vi "Main.vi"() -> ()   [LabVIEW 2019]
doc: "The myRIO Project template acquires acceleration data from the onboard accelerometer and displays the changes of acceleration values in a waveform chart."
uses:
  <vilib>/myRIO/Common/Instrument Driver Framework/myRIO v1.0/Encoder/typedefs/Encoder Count Direction Enum.ctl
  <vilib>/myRIO/Common/Instrument Driver Framework/myRIO v1.0/Encoder/typedefs/Encoder Signal Mode.ctl
  <vilib>/myRIO/Common/Instrument Driver Framework/myRIO v1.0/Encoder/typedefs/Encoder Channels Enum.ctl
  <vilib>/myRIO/Common/Instrument Driver Framework/Utilities/typedefs/Generic FPGA Reference.ctl
  <vilib>/myRIO/Common/Instrument Driver Framework/Utilities/typedefs/myRIO v1.0 Reference.ctl
  <vilib>/myRIO/Common/Instrument Driver Framework/Utilities/typedefs/Hardware Version Enum.ctl
  <vilib>/myRIO/Common/Instrument Driver Framework/Utilities/typedefs/myRIO Generic Hardware Reference.ctl
  <vilib>/myRIO/Instrument Drivers/Onboard IO/Encoder/typedefs/Encoder Reference.ctl
  <vilib>/myRIO/Instrument Drivers/Onboard IO/Encoder/Encoder.lvlib
  <vilib>/myRIO/Instrument Drivers/Onboard IO/Encoder/vis/Read.vi
  <vilib>/myRIO/Common/Instrument Driver Framework/myRIO v1.0/Encoder/typedefs/Encoder Configuration v1.0.ctl
  <vilib>/userDefined/High Color/nirio_resource_hc.ctl
  <vilib>/myRIO/Common/Instrument Driver Framework/myRIO v1.0/Encoder/vis/myRIO v1.1 Open Encoder.vi
  <vilib>/myRIO/Common/Instrument Driver Framework/myRIO v1.0/Encoder/vis/myRIO v1.0 Configure Encoder.vi
  <vilib>/myRIO/Instrument Drivers/Onboard IO/Encoder/vis/myRIO Encoder Open.xnode
  <vilib>/myRIO/Common/Instrument Driver Framework/Utilities/vis/Is FPGA Ref Available.vi
  <vilib>/myRIO/Express VI/Onboard IO/Encoder/Encoder Express VI.xnode
  <vilib>/ptbypt/NI_PtbyPt.lvlib
  <vilib>/myRIO/Instrument Drivers/Onboard IO/PWM/typedefs/PWM Configuration.ctl
  <vilib>/myRIO/Instrument Drivers/Onboard IO/PWM/PWM.lvlib
  <vilib>/myRIO/Common/Instrument Driver Framework/myRIO v1.0/PWM/typedefs/PWM Channels Enum.ctl
  <vilib>/myRIO/Instrument Drivers/Onboard IO/PWM/typedefs/PWM Reference.ctl
  <vilib>/myRIO/Instrument Drivers/Onboard IO/PWM/vis/Set Duty Cycle and Frequency.vi
  <vilib>/myRIO/Common/Instrument Driver Framework/myRIO v1.0/PWM/vis/myRIO v1.1 Open PWM.vi
  <vilib>/myRIO/Instrument Drivers/Onboard IO/PWM/vis/myRIO PWM Open.xnode
  <vilib>/myRIO/Express VI/Onboard IO/PWM/PWM Express VI.xnode
  <vilib>/myRIO/Common/Instrument Driver Framework/myRIO v1.0/DIO/typedefs/DIO Channels Enum.ctl
  <vilib>/myRIO/Common/Instrument Driver Framework/myRIO v1.0/DIO/typedefs/DIO Channels List.ctl
  <vilib>/myRIO/Instrument Drivers/Onboard IO/DIO/typedefs/DIO Reference.ctl
  <vilib>/myRIO/Instrument Drivers/Onboard IO/DIO/DIO.lvlib
  <vilib>/myRIO/Instrument Drivers/Onboard IO/DIO/vis/Write.vi
  <vilib>/myRIO/Common/Instrument Driver Framework/myRIO v1.0/DIO/vis/myRIO v1.1 Open DIO.vi
  <vilib>/myRIO/Instrument Drivers/Onboard IO/DIO/vis/myRIO DIO Open.xnode
  <vilib>/myRIO/Express VI/Onboard IO/DO/DO Express VI.xnode
  <vilib>/addons/control/pid/NI_PID_pid.lvlib
  <vilib>/addons/control/pid/pid.llb/PID (DBL).vi
  <vilib>/myRIO/Common/Instrument Driver Framework/myRIO v1.0/Accelerometer/typedefs/Accelerometer Channels Enum.ctl
  <vilib>/myRIO/Common/Instrument Driver Framework/myRIO v1.0/Accelerometer/typedefs/Accelerometer Channels List.ctl
  <vilib>/myRIO/Instrument Drivers/Onboard Devices/Accelerometer/typedefs/Accelerometer Reference.ctl
  <vilib>/myRIO/Instrument Drivers/Onboard Devices/Accelerometer/Accelerometer.lvlib
  <vilib>/myRIO/Instrument Drivers/Onboard Devices/Accelerometer/vis/Read.vi
  <vilib>/myRIO/Instrument Drivers/Onboard Devices/Accelerometer/vis/myRIO Accelerometer Open.xnode
  <vilib>/myRIO/Express VI/Onboard Devices/Accelerometer/Accelerometer Express VI.xnode
  <vilib>/myRIO/Instrument Drivers/Utilities/Utilities.lvlib
  <vilib>/Utility/file.llb/Write Delimited Spreadsheet (DBL).vi
  <vilib>/myRIO/Common/Instrument Driver Framework/myRIO v1.0/Accelerometer/vis/myRIO v1.1 Open Accelerometer.vi
panel:
  out "Velocidad M2":dbl
  out "Velocidad  M1":dbl
  out "Aporte de FF-M1":dbl
  out "Aporte de FF-M2":dbl
  out "Distancia M2":dbl
  out "Distancia  M1":dbl
  in  "T pasa-bajos":dbl=0.1
  in  "zona_muerta (°)":dbl=2.5
  out "aX_grav":dbl
  in  "KgR_sub":dbl=0.18 format="%#_13g"
  in  "KgR_baj":dbl=0.11 format="%#_13g"
  in  "KgL_baj":dbl=0.12 format="%#_13g"
  in  "KgL_sub":dbl=0.19 format="%#_13g"
  in  "Offset acel_X":dbl=-0.114
  in  "ang_rampa":dbl=10.0
  out "Inclinación X":dbl
  in  "Offset_acel_Y":dbl
  out "Inclinación Y":dbl
  out "Duty Cycle calculado":dbl
  out "Duty Cycle enviado":dbl
  out "roll_n":dbl
  out "pitch_n":dbl
  out "Verifica si se guardo csv":errorcluster
  out "Verifica si se guardo csv 2":errorcluster
  out "error out 2":errorcluster
  out "RPM M1":dbl
  out "RPM GAUGE M1":dbl(knob) scale=0.0..100.0
  out "Dirección de Giro M1":enum16{"Counting Up", "Counting Down"}(ring)
  out "Cuentas M1 (Der)":dbl
  out "Posición angular M1":dbl(knob) scale=-360.0..360.0
  out "Posición M1":dbl
  out "Frecuencia (rev/s)":dbl
  out "Vueltas Dadas M1":dbl
  out "Posición angular M2":dbl(knob) scale=-360.0..360.0
  out "Dirección de Giro M2":enum16{"Counting Up", "Counting Down"}(ring)
  out "Posición M2":dbl
  out "RPM GAUGE M2":dbl(knob) scale=0.0..100.0
  out "Vueltas Dadas M2":dbl
  out "RPM M2":dbl
  out "Cuentas M2 (Izq)":dbl
  in  "Referencia M1 y M2":dbl
  in  "Velocidad":dbl
  in  "v(cm/s)":dbl
  in  "w (rad/s)":dbl
  in  "PWM Manual":dbl
  out "a_encoder":dbl
  out "a_enc_f":dbl
  out "aX_f":dbl
  out "aY_f":dbl
  out "aZ_f":dbl
  out "phi":dbl
  out "phi_deg":dbl
  out "periodo real (seg)":dbl
  in  "Ref Platfform Movement":dbl
  in  "ROBOT MÓVIL CON PLATAFORMA DE BALANCEO - GRUPO 2":T1(tab)
  in  "?":bool
  in  "Tipo de referencia":enum16{"Sinusoidal", "Constante"}(ring)
  out "Coordenada xy vs t":cluster{dbl, dbl, "Referencia":dbl}(graph)
  out "Angulos de servos":cluster{dbl, dbl}(graph)
  out "Recepción del UART":string
  in  "PID EJE Y":T2={"proportional gain (Kc)"=0.14897, "integral time (Ti, min)"=0.03, "derivative time (Td, min)"=0.004327} {"derivative time (Td, min)" format="%.6f"; "integral time (Ti, min)" format="%.6f"; "proportional gain (Kc)" format="%.6f"}
  in  "PID EJE X":T2={"proportional gain (Kc)"=0.1164, "integral time (Ti, min)"=0.03, "derivative time (Td, min)"=0.005282} {"derivative time (Td, min)" format="%.6f"; "integral time (Ti, min)" format="%.6f"; "proportional gain (Kc)" format="%.6f"}
  in  "Frecuencia (Hz)":dbl=50.0
  in  "Modo de operación":enum16{"Platform movement", "Ball Control"}(ring)=enum."Ball Control"
  in  "dt (s)":dbl=0.0167 format="%.4f"
  in  "Tipo de control":enum16{"SMC", "LQR", "PID"}(ring)=enum."PID"
  in  "Eje":enum16{"xy", "y", "x", "Home"}(ring)
  in  "Referencia Control":dbl
  in  "Rango Salida Y":cluster{"output high":dbl, "output low":dbl}={"output high"=25.0, "output low"=-25.0} {"output low" format="%.2f"; "output high" format="%.2f"}
  in  "Rango Salida X":cluster{"output high":dbl, "output low":dbl}={"output high"=25.0, "output low"=-25.0} {"output low" format="%.2f"; "output high" format="%.2f"}
  out "Saturación (inclinación de plataforma)":cluster{dbl, dbl}(graph)
  in  "Longitud de brazo [mm]":dbl=35.0
  in  "R (L/2) [mm]":dbl=59.0
  out "Roll -  Eje X":dbl
  out "Pitch - Eje Y":dbl
  out "Error Ángulo (°)":dbl
  out "Error Distancia (cm)":dbl
  out "LLEGÓ":bool
  out "Avanzando":bool
  out "Girando":bool
  in  "Tolerancia (cm)":dbl=0.3
  out "Recorrido Eje X (cm)":dbl
  out "SIGUE Vel M2":bool
  out "SIGUE Vel M1":bool
  out "Comportamiento de ángulos (°)":cluster{"phi_lim":dbl, "roll_lim":dbl}(graph)
  out "Control Lazo Interno":cluster{"f":dbl, dbl, "f":dbl, dbl}(graph)
  in  "Movimiento":T3(ring)=enum."Recta"
  in  "INICIAR MOTORES":bool
  in  "STOP ALL":bool
  in  "Referencia":dbl=220.0
  in  "REINICIAR":bool caption="Reiniciar cuentas"
  in  "PI - M1":T2={"proportional gain (Kc)"=0.014853, "integral time (Ti, min)"=0.000665, "derivative time (Td, min)"=0.0} {"derivative time (Td, min)" format="%.6f"; "integral time (Ti, min)" format="%.6f"; "proportional gain (Kc)" format="%.6f"}
  in  "PI - M2":T2={"proportional gain (Kc)"=0.01026, "integral time (Ti, min)"=0.000604, "derivative time (Td, min)"=0.0} {"derivative time (Td, min)" format="%.6f"; "integral time (Ti, min)" format="%.6f"; "proportional gain (Kc)" format="%.6f"}
  out "Señal de control de Velocidades":cluster{"output":dbl, "output":dbl}(graph)
  out "Lazo externo - Posición":cluster{"x":dbl, "y":dbl}(graph)={"x"=50.0, "y"=49.66663306165075}
  out "Lazo externo - Rumbo":cluster{"x":dbl, "y":dbl}(graph)
  in  "MODO CONTROL":T4(ring)=enum."Trayectoria"
  out "Móvil dt":dbl=0.01
  out "X (cm)":dbl
  out "Y (cm)":dbl
  out "theta (deg)":dbl
  in  "Kd":dbl=1.38 format="%#_13g"
  in  "Ky":dbl=0.048 format="%#_13g"
  in  "Kth":dbl=1.38 format="%#_13g"
  in  "Tol cm/s":dbl=1.5
  out "Falla M2":bool
  out "Falla M1":bool
  in  "Rango Salida PWM":cluster{"output high":dbl, "output low":dbl}={"output high"=1.0, "output low"=-1.0} {"output low" format="%.2f"; "output high" format="%.2f"}
  out "Desvio en Y (cm)":cluster{"y":dbl}(graph)
  out "Giro Realizado (°)":dbl
  # "Filtro Pasa - Bajo"
  # "Lectura - Lazo Interno"
  # "Lectura - Lazo Externo"
  # "Feed-Forward"
  # "CONTROL PID DE CADA EJE -  PLATAFORMA DE BALANCEO"
  # "Reinicio"
  # "CONTROL DE TRAYECTORIA EN CASCADA - BASE MÓVIL"
  # "Operación y Seguridad"
  # "Modo de Control - Lazo Interno"
  # "Modo de Control - Lazo Externo"
  # "ODOMETRÍA"
  # "GANANCIAS - LAZO EXTERNO"
  # "ERROR Y LLEGADA"
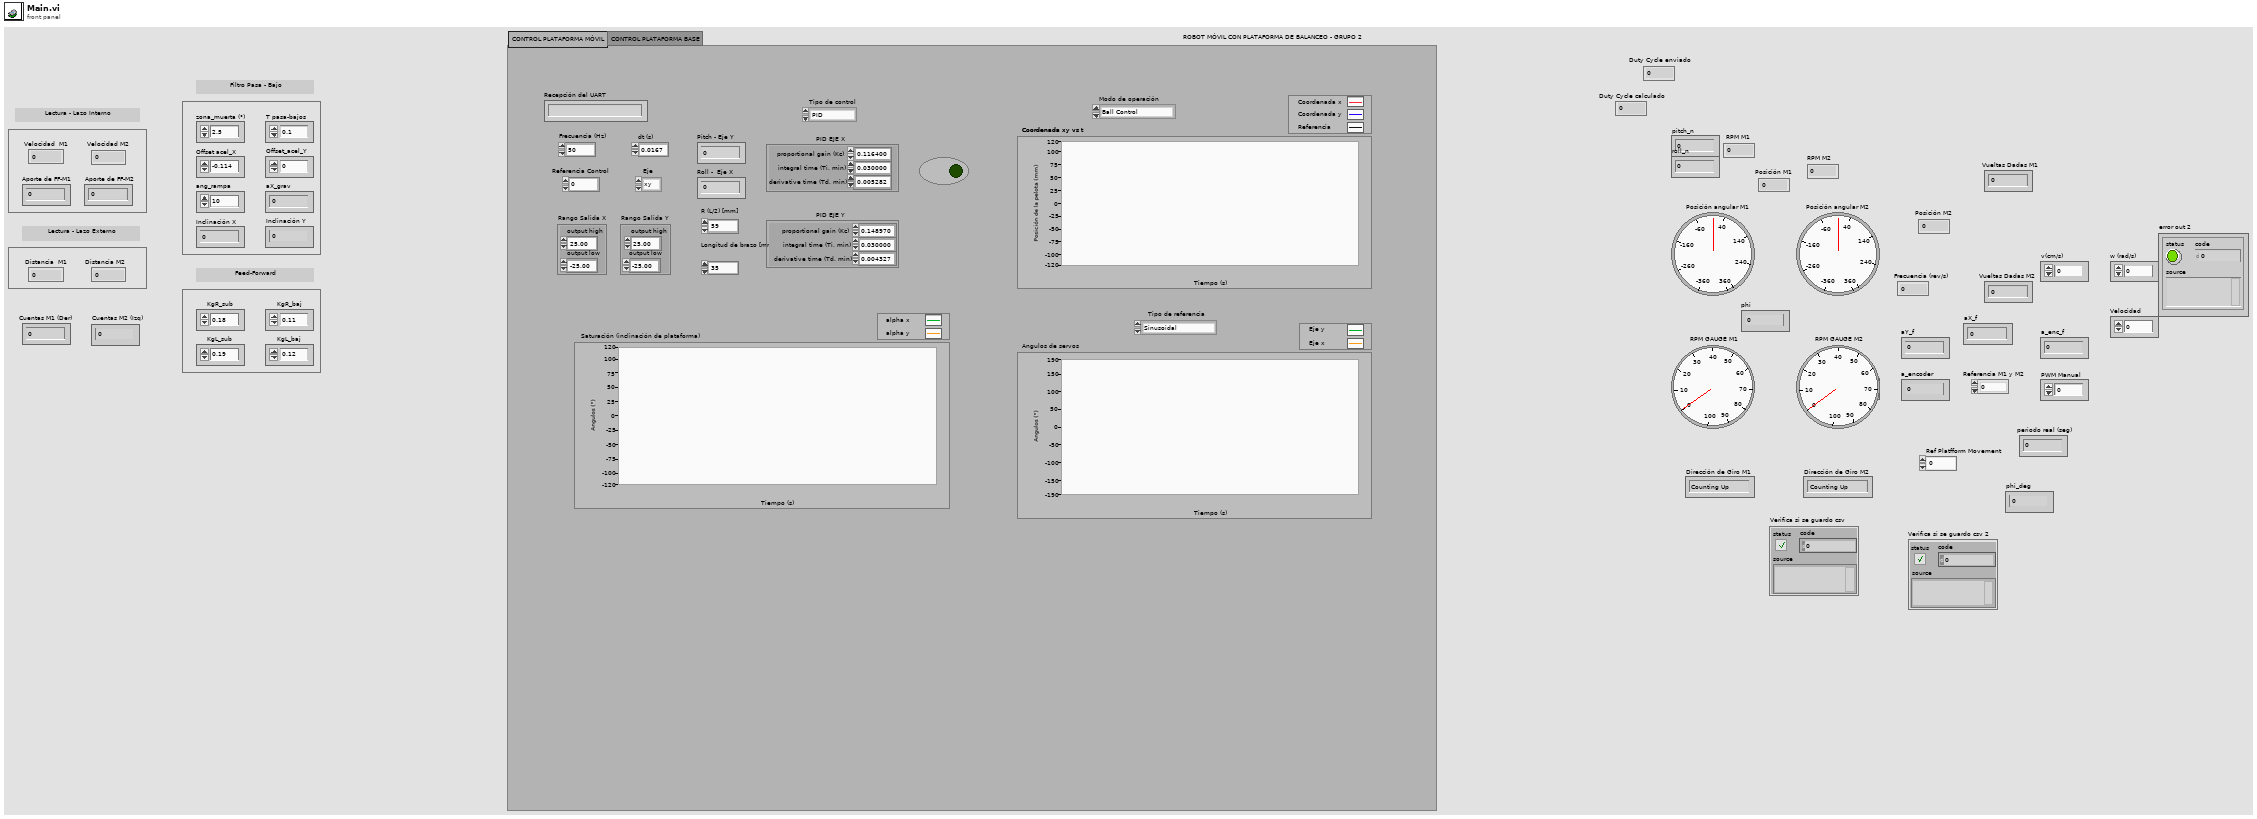
[diagram p1: front panel]
types:
  T1 = enum32{"CONTROL PLATAFORMA MÓVIL", "CONTROL PLATAFORMA BASE"}
  T2 = cluster{"proportional gain (Kc)":dbl, "integral time (Ti, min)":dbl, "derivative time (Td, min)":dbl}
  T3 = enum16{"Manual", "Recta", "Giro centro", "Giro rueda fija", "Rutina Piso", "Ida y Vuelta", "Rutina Rampa", ""}
  T4 = enum16{"Identificación", "Lazo Interno", "Trayectoria"}
  T5 = typedef "PWM.lvlib/PWM Reference.ctl" = cluster{"myRIO Reference":T6, "PWM Channels Enum":T10, "PWM Configuration":T11}
  T6 = typedef "myRIO Generic Hardware Reference.ctl" = cluster{"myRIO Model":T7, "myRIO Hardware Reference":T8}
  T7 = typedef "Hardware Version Enum.ctl" = enum16{"Unknown", "myRIO-1900", "myRIO-1950", "roboRIO", "NI ELVIS RIO CM", "ELVIS III"}
  T8 = typedef "myRIO v1.0 Reference.ctl" = cluster{"Generic FPGA Reference":T9, "Allow multiple opens":bool}
  T9 = typedef "Generic FPGA Reference.ctl" = refnum<k20>
  T10 = typedef "PWM Channels Enum.ctl" = enum16{"Not Connected", "C/PWM0", "C/PWM1", "A/PWM0", "A/PWM1", "A/PWM2", "A/PWM3", "A/PWM4", "A/PWM5", "A/PWM6", "A/PWM7", "A/PWM8", "A/PWM9", "A/PWM10", "A/PWM11", "A/PWM12", "A/PWM13", "A/PWM14", "A/PWM15", "A/PWM16", "A/PWM17", "A/PWM18", "A/PWM19", "B/PWM0", "B/PWM1", "B/PWM2", "B/PWM3", "B/PWM4", "B/PWM5", "B/PWM6", "B/PWM7", "B/PWM8", "B/PWM9", "B/PWM10", "B/PWM11", "B/PWM12", "B/PWM13", "B/PWM14", "B/PWM15", "B/PWM16", "B/PWM17", "B/PWM18", "B/PWM19", "PWM/PWM0", "PWM/PWM1", "PWM/PWM2", "PWM/PWM3", "PWM/PWM4", "PWM/PWM5", "PWM/PWM6", "PWM/PWM7", "PWM/PWM8", "PWM/PWM9"}
  T11 = typedef "PWM.lvlib/PWM Configuration.ctl" = cluster{"Frequency":dbl, "Duty Cycle":dbl}
  T12 = typedef "nirio_resource_hc.ctl" = tag
  T13 = enum16{"Identificación", "Lazo Interno", "Trayectoria", ""}
  T14 = typedef "Accelerometer.lvlib/Accelerometer Reference.ctl" = cluster{"myRIO Reference":T6, "Accelerometer Channels List":T15, "LSB Weight":dbl}
  T15 = typedef "Accelerometer Channels List.ctl" = T16[]
  T16 = typedef "Accelerometer Channels Enum.ctl" = enum16{"Not Connected", "X-Axis", "Y-Axis", "Z-Axis"}
  T17 = typedef "DIO.lvlib/DIO Reference.ctl" = cluster{"myRIO Reference":T6, "DIO Channels List":T18}
  T18 = typedef "DIO Channels List.ctl" = T19[]
  T19 = typedef "DIO Channels Enum.ctl" = enum16{"Not Connected", "C/DIO0", "C/DIO1", "C/DIO2", "C/DIO3", "C/DIO4", "C/DIO5", "C/DIO6", "C/DIO7", "A/DIO0", "A/DIO1", "A/DIO2", "A/DIO3", "A/DIO4", "A/DIO5", "A/DIO6", "A/DIO7", "A/DIO8", "A/DIO9", "A/DIO10", "A/DIO11", "A/DIO12", "A/DIO13", "A/DIO14", "A/DIO15", "A/DIO16", "A/DIO17", "A/DIO18", "A/DIO19", "B/DIO0", "B/DIO1", "B/DIO2", "B/DIO3", "B/DIO4", "B/DIO5", "B/DIO6", "B/DIO7", "B/DIO8", "B/DIO9", "B/DIO10", "B/DIO11", "B/DIO12", "B/DIO13", "B/DIO14", "B/DIO15", "B/DIO16", "B/DIO17", "B/DIO18", "B/DIO19", "LED0", "LED1", "LED2", "LED3", "Button0", "DIO/DIO0", "DIO/DIO1", "DIO/DIO2", "DIO/DIO3", "DIO/DIO4", "DIO/DIO5", "DIO/DIO6", "DIO/DIO7", "DIO/DIO8", "DIO/DIO9", "SPI/CS0", "SPI/CS1", "SPI/CS2", "SPI/CS3", "LED RADIO (Green)", "LED RADIO (Red)", "LED COMM (Green)", "LED COMM (Red)", "LED MODE (Green)", "LED MODE (Red)"}
  T20 = typedef "Encoder.lvlib/Encoder Reference.ctl" = cluster{"myRIO Reference":T6, "Encoder Channels Enum":T21}
  T21 = typedef "Encoder Channels Enum.ctl" = enum16{"Not Connected", "C/ENC0", "C/ENC1", "A/ENC", "A/ENC0", "A/ENC1", "A/ENC2", "A/ENC3", "A/ENC4", "A/ENC5", "A/ENC6", "A/ENC7", "A/ENC8", "A/ENC9", "B/ENC", "B/ENC0", "B/ENC1", "B/ENC2", "B/ENC3", "B/ENC4", "B/ENC5", "B/ENC6", "B/ENC7", "B/ENC8", "B/ENC9", "DIO/ENC0", "DIO/ENC1", "DIO/ENC2", "DIO/ENC3", "DIO/ENC4"}
  T22 = typedef "Encoder Signal Mode.ctl" = enum16{"Quadrature phase signal", "Step and direction signal"}
  T23 = enum16{"open", "replace", "create", "open or create", "replace or create", "replace or create with confirmation"}
  T24 = typedef "Encoder Count Direction Enum.ctl" = enum16{"Counting Up", "Counting Down"}
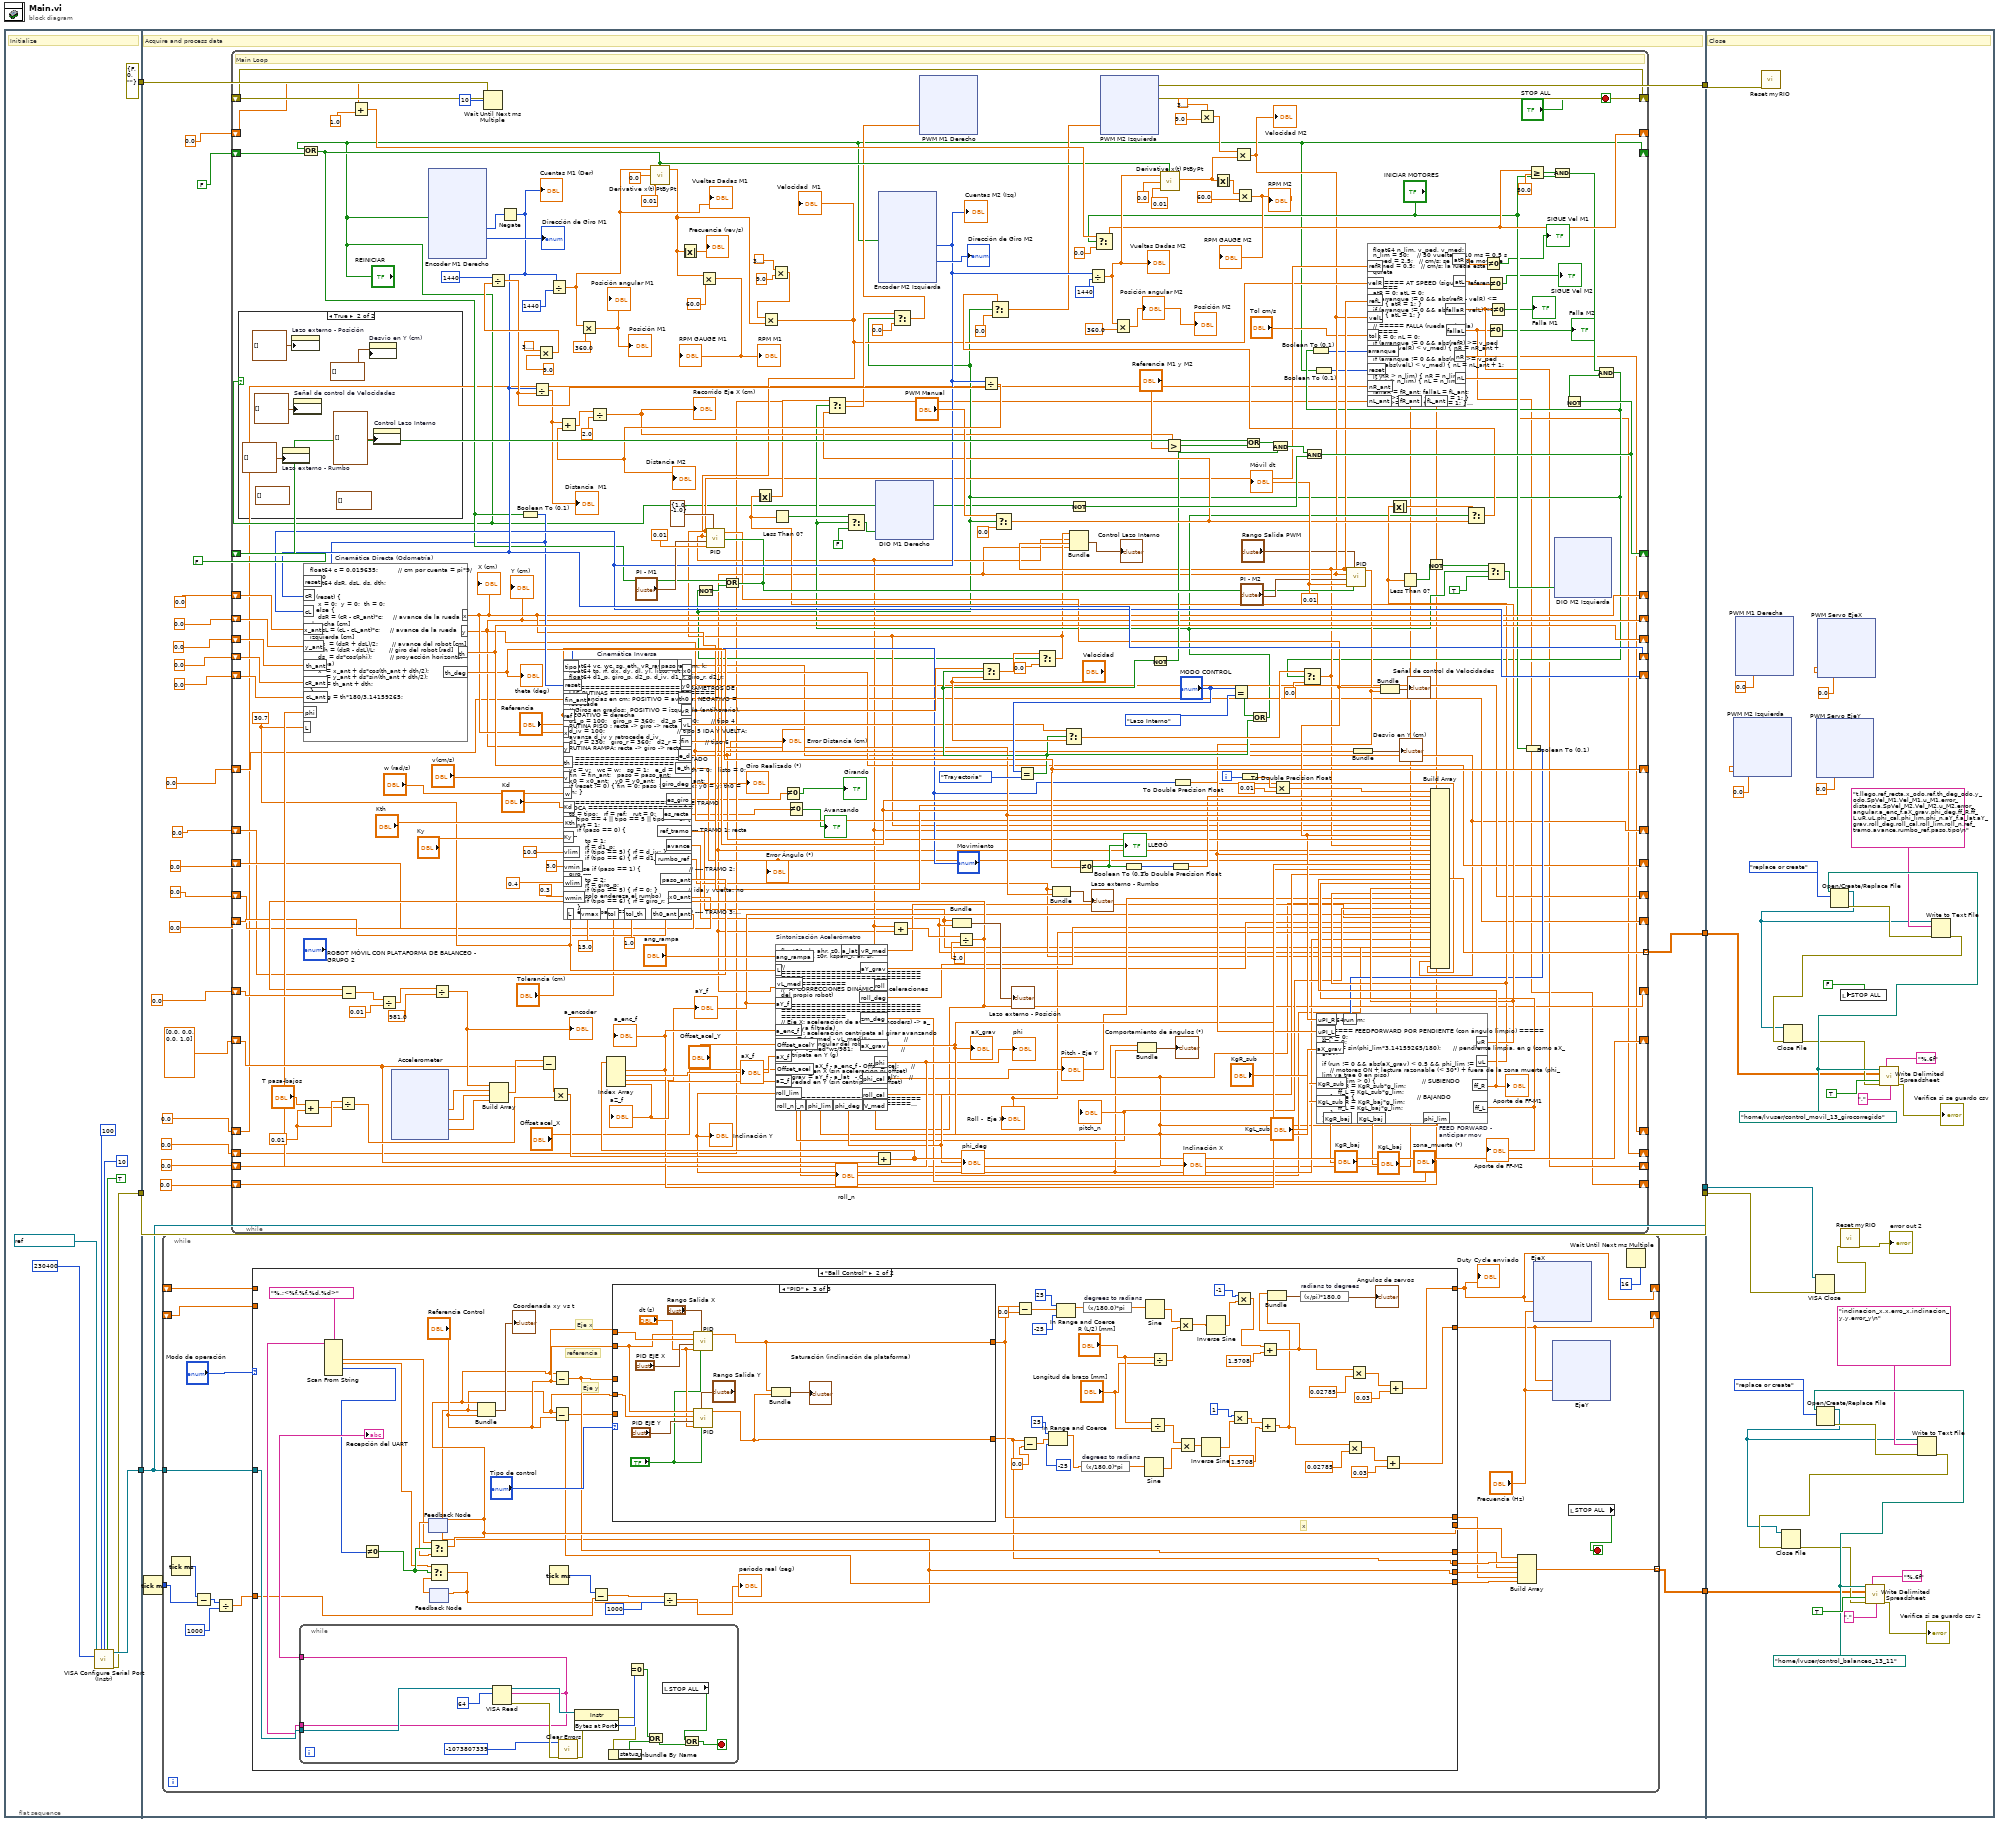
[diagram p0: block diagram]
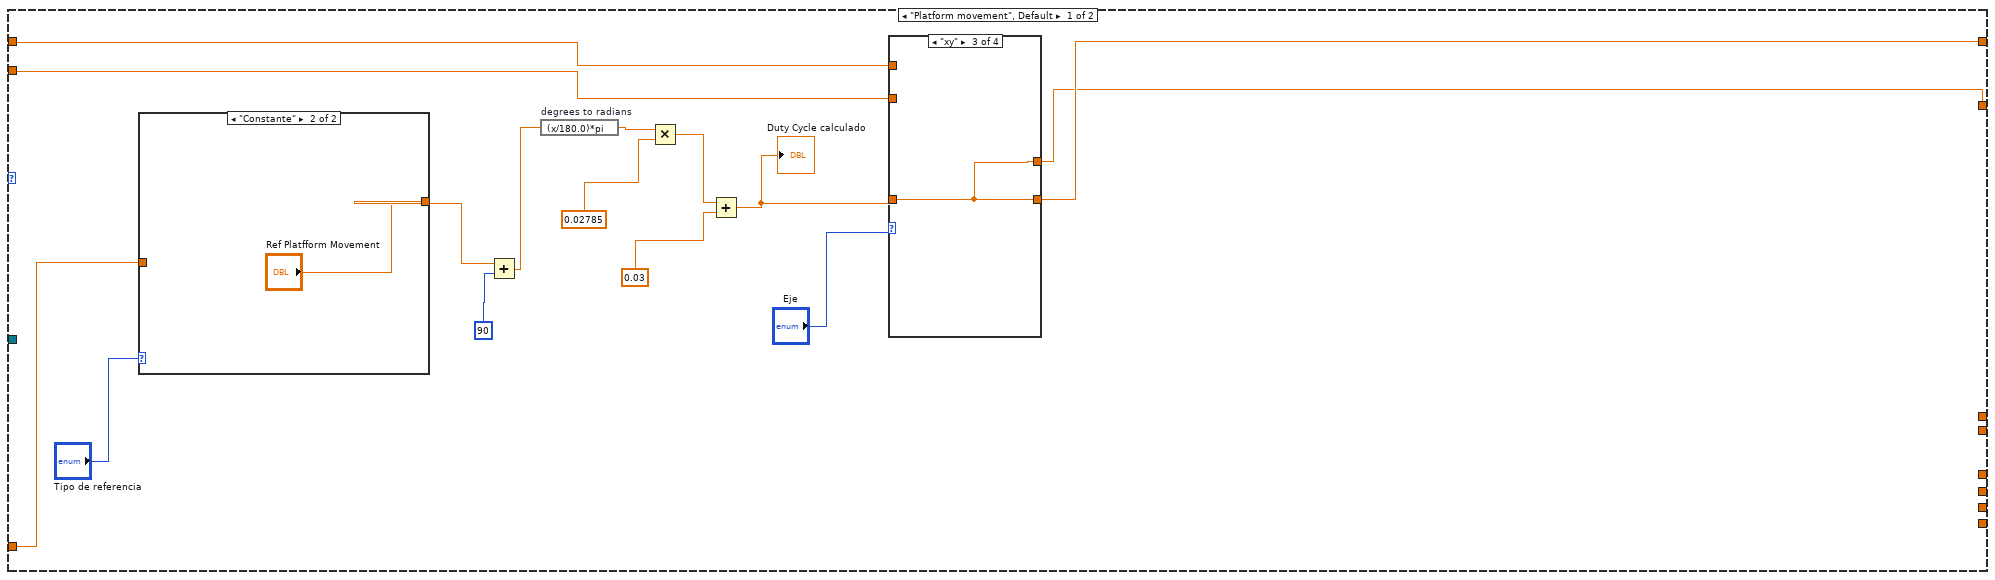
[diagram p2: hidden frame]
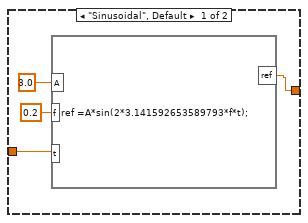
[diagram p3: hidden frame]
diagram:
  n1 = flat-sequence {
    tunnel: [errorcluster {"status"=FALSE, "code"=0, "source"=""} ("error in (no error)")] -> w8
    tunnel: [w10] -> w7
    tunnel: [w9] -> w6
    tunnel: w8 -> [w42]
    tunnel: [w41] -> w5
    tunnel: [w29] -> w4
    tunnel: w7 -> [w25]
    tunnel: [w27] -> w3
    tunnel: w6 -> [w26]
    tunnel: [w26] -> w2
    tunnel: [w25] -> w1
    tunnel: w5 -> [w802]
    tunnel: w4 -> [w786]
    tunnel: w3 -> [w774]
    tunnel: w2 -> [w771]
    tunnel: w1 -> [w770]
    frame #0 {
      # "Initialize"
      n2 = call <vilib>:"VISA Configure Serial Port (Instr).vi"("VISA resource name"=refnum<visa-resource-name> "ASRL1::INSTR", "timeout (10sec)"=u32 100, "termination char\n(0xA = '\\n' = LF)"=u8 10 ("termination char\n(0xA = '\\n' = LF)"), "Enable Termination\nChar (T)"=TRUE ("Enable Termination\nChar (T)"), "baud rate (9600)"=u32 230400) -> ("VISA resource name out"=w10:refnum<visa-resource-name>, "error out"=w9:errorcluster)  [unwired: 9 in]
    }
    frame #1 {
      # "Acquire and process data"
      n3 = Tick Count (ms)() -> (millisecond timer value=w28:u32)
      n4 = while {
        shift-right: [w58] -> _
        shift-left: _ -> [w62]
        shift-right: [w59] -> _
        shift-left: _ -> [w61]
        tunnel: w25 -> [w57]
        tunnel: w28 -> [w51]
        tunnel: [w44] -> w27 mode=indexing
        stop <- w43 stop-if-true
        n5 = Tick Count (ms)() -> (millisecond timer value=w55:u32)
        n6 = Subtract(x=w55, y=w51) -> (x-y=w54:u32)
        n7 = Divide(x=w54, y=u32 1000) -> (x/y=w52:dbl)
        n8 = case shown="\"Ball Control\"" "Modo de operación" {
          tunnel: w62 -> [w143 _]
          tunnel: w61 -> [w142 _]
          tunnel: [w141 w213] -> w58
          tunnel: [w140 w212] -> w59
          tunnel: w57 -> [_ w190]
          tunnel: w52 -> [w134 w172]
          tunnel: [_ w170] -> w50
          tunnel: [_ w163] -> w49
          tunnel: [_ w169] -> w48
          tunnel: [_ w167] -> w47
          tunnel: [_ w165] -> w46
          tunnel: [_ w168] -> w45
          frame "Platform movement", Default {
            n9 = case shown="\"Constante\"" "Tipo de referencia" {
              tunnel: [w152 "Ref Platfform Movement"] -> w135
              tunnel: w134 -> [w149 _]
              frame "Sinusoidal", Default {
                n10 = formula code="ref =A*sin(2*3.141592653589793*f*t);"("A"=3.0 ("input variable"), "f"=0.2 ("input variable"), "t"=w149) -> ("ref"=w152:dbl)
              }
              frame "Constante" {
              }
            }
            n11 = Add(x=w135, y=90) -> (x+y=w138:dbl)
            n12 = expression code="(x/180.0)*pi" "degrees to radians"(w138) -> (w145:dbl)
            n13 = Multiply(x=w145, y=0.02785 ("ax")) -> (x*y=w146:dbl)
            n14 = Add(x=w146, y=0.03 ("ax")) -> (x+y=w144:dbl)
            "Duty Cycle calculado" <- w144
            n15 = case shown="\"xy\"" "Eje" {
              tunnel: w144 -> [w154 w157 w158 _]
              tunnel: w143 -> [w155 _ _ w160]
              tunnel: w142 -> [_ w156 _ w159]
              tunnel: [w155 w157 w158 w160] -> w141
              tunnel: [w154 w156 w158 w159] -> w140
              frame "y", Default {
              }
              frame "x" {
              }
              frame "xy" {
              }
              frame "Home" {
              }
            }
          }
          frame "Ball Control" {
            # "x"
            # "Eje y"
            # "Eje x"
            # "referencia"
            n16 = while {
              tunnel: w190 -> [w238]
              tunnel: [w228] -> w189
              tunnel: [w228] -> w188
              stop <- w225 stop-if-true
              n17 = VISA Read(VISA resource name=w238, byte count=u32 64) -> (VISA resource name out=w233:refnum<visa-resource-name>, read buffer=w228:string, error out=w236:errorcluster)  [unwired: 1 in, 1 out]
              n18 = call <vilib>:"Clear Errors.vi"("error in (no error)"=w236, "specific error code to clear (0: all)"=-1073807339) -> ("error out"=w234:errorcluster)  [unwired: 4 in, 1 out]
              n19 = property on="Property Node" class="Instr"(reference=w233, error in=w234) -> (error out=w231:errorcluster, "Bytes at Port"=w232:u32)  [unwired: 1 out]
              n20 = Unbundle By Name(w231) -> ("status"=w229:bool)
              n21 = Equal To 0?(x=w232) -> (x = 0?=w230:bool)
              n22 = Or(x=w230, y=w229) -> (x .or. y?=w227:bool)
              n23 = local read "STOP ALL"() -> (w226:bool)
              n24 = Or(x=w226, y=w227) -> (x .or. y?=w225:bool)
            }
            "Recepción del UART" <- w188
            n25 = Scan From String(format string="%.;<%f,%f,%d,%d>", input string=w189) -> (output 1=w182:dbl, output 2=w181:dbl, output 3=w179:i32)  [unwired: 7 in, 3 out]
            n26 = Not Equal To 0?(x=w179) -> (x != 0?=w184:bool)
            n27 = feedback #1() -> (w183:dbl)  [unwired: 1 in]
            n28 = feedback #2() -> (w180:dbl)  [unwired: 1 in]
            n29 = Select(t=w181, s=w184, f=w180) -> (s? t:f=w167:dbl)
            n30 = feedback-in #2(w167) -> ()
            n31 = Select(t=w182, s=w184, f=w183) -> (s? t:f=w170:dbl)
            n32 = feedback-in #1(w170) -> ()
            n33 = Bundle(w170, w167, "Referencia Control"="Referencia Control") -> (→"Coordenada xy vs t":cluster{dbl, dbl, "Referencia Control":dbl})  [unwired: 1 in]
            n34 = Tick Count (ms)() -> (millisecond timer value=w171:u32)
            n35 = Subtract(x=w167, y="Referencia Control") -> (x-y=w168:dbl)
            n36 = Subtract(x=w170, y="Referencia Control") -> (x-y=w169:dbl)
            n37 = Subtract(x=w171, y=w172) -> (x-y=w175:dbl)
            n38 = case shown="\"PID\"" "Tipo de control" {
              tunnel: w169 -> [w239 w241 _]
              tunnel: w168 -> [_ _ _]
              tunnel: [w240 w242 w248] -> w165
              tunnel: [w239 w241 w247] -> w163
              tunnel: w170 -> [w240 w242 w254]
              tunnel: "Referencia Control" -> [_ _ w252]
              tunnel: w167 -> [_ _ w251]
              frame "SMC", Default {
              }
              frame "LQR" {
              }
              frame "PID" {
                n39 = call-poly <vilib>:"PID.vi"("reinitialize? (F)"="?", "output range"="Rango Salida X", "dt (s)"="dt (s)", "PID gains"="PID EJE X", "process variable"=w254, "setpoint"=w252) -> ("output"=w248:dbl)  [unwired: 4 in, 1 out]
                n40 = call-poly <vilib>:"PID.vi"("reinitialize? (F)"="?", "output range"="Rango Salida Y", "dt (s)"="dt (s)", "PID gains"="PID EJE Y", "process variable"=w251, "setpoint"=w252) -> ("output"=w247:dbl)  [unwired: 4 in, 1 out]
                n41 = Bundle("output"=w248, "output"=w247) -> (→"Saturación (inclinación de plataforma)":cluster{"output":dbl, "output":dbl})  [unwired: 1 in]
              }
            }
            n42 = Divide(x=w175, y=u32 1000) -> (x/y=→"periodo real (seg)":dbl)
            n43 = Subtract(x=w165, y=0.0) -> (x-y=w166:dbl)
            n44 = Subtract(x=w163, y=0.0) -> (x-y=w164:dbl)
            n45 = In Range and Coerce(upper limit=25, x=w164, lower limit=-25) -> (coerced(x)=w196:dbl)  [unwired: 1 out]
            n46 = In Range and Coerce(upper limit=25, x=w166, lower limit=-25) -> (coerced(x)=w198:dbl)  [unwired: 1 out]
            n47 = expression code="(x/180.0)*pi" "degrees to radians"(w196) -> (w197:dbl)
            n48 = expression code="(x/180.0)*pi" "degrees to radians"(w198) -> (w199:dbl)
            n49 = Sine(x=w197) -> (sin(x)=w202:dbl)
            n50 = Sine(x=w199) -> (sin(x)=w209:dbl)
            n51 = Divide(x="R (L/2) [mm]", y="Longitud de brazo [mm]") -> (x/y=w201:dbl)
            n52 = Divide(x="R (L/2) [mm]", y="Longitud de brazo [mm]") -> (x/y=w208:dbl)
            n53 = Multiply(x=w209, y=w208) -> (x*y=w207:dbl)
            n54 = Multiply(x=w201, y=w202) -> (x*y=w200:dbl)
            n55 = Inverse Sine(1:w200) -> (0:w186:dbl)
            n56 = Inverse Sine(1:w207) -> (0:w176:dbl)
            n57 = Multiply(x=1, y=w186) -> (x*y=w187:dbl)
            n58 = Multiply(x=-1, y=w176) -> (x*y=w177:dbl)
            n59 = Add(x=w187, y=1.5708) -> (x+y=w191:dbl)
            n60 = Add(x=w177, y=1.5708) -> (x+y=w192:dbl)
            n61 = Bundle(w191, w192) -> (w193:cluster{dbl, dbl})  [unwired: 1 in]
            n62 = expression code="(x/pi)*180.0" "radians to degrees"(w193) -> (→"Angulos de servos":cluster{dbl, dbl})
            n63 = Multiply(x=w191, y=0.02785 ("ax")) -> (x*y=w221:dbl)
            n64 = Multiply(x=w192, y=0.02785 ("ax")) -> (x*y=w218:dbl)
            n65 = Add(x=w221, y=0.03 ("ax")) -> (x+y=w212:dbl)
            n66 = Add(x=w218, y=0.03 ("ax")) -> (x+y=w213:dbl)
          }
        }
        "Duty Cycle enviado" <- w58
        n67 = Build Array(w50, w49, w48, w47, w46, w45) -> (w44:dbl[])
        n68 = xnode ("EjeX")("Duty Cycle"=w58, "Frequency [Hz]"="Frecuencia (Hz)") -> ()  [unwired: 1 in, 1 out]
        n69 = xnode ("EjeY")("Duty Cycle"=w59, "Frequency [Hz]"="Frecuencia (Hz)") -> ()  [unwired: 1 in, 1 out]
        n70 = local read "STOP ALL"() -> (w43:bool)
        n71 = Wait Until Next ms Multiple(millisecond multiple=u32 16 ("milliseconds to wait")) -> ()  [unwired: 1 out]
      }
      n72 = while {
        shift-right: [w492] -> w41
        shift-left: w42 -> [w492]
        shift-right: [w449] -> _
        shift-left: FALSE -> [w459]
        shift-right: [w446] -> _
        shift-left: 0.0 -> [w452]
        shift-right: [w350] -> _
        shift-left: 0.0 -> [w427]
        shift-right: [w340] -> _
        shift-left: 0.0 -> [w358]
        shift-right: [w395] -> _
        shift-left: 0.0 -> [w426]
        shift-right: [w408] -> _
        shift-left: 0.0 -> [w425]
        shift-right: [w407] -> _
        shift-left: 0.0 -> [w424]
        shift-right: ["REINICIAR"] -> _
        shift-left: FALSE -> [w277]
        shift-right: [w388] -> _
        shift-left: 0.0 -> [w300]
        shift-right: [w315] -> _
        shift-left: 0.0 -> [w373]
        shift-right: [w357] -> _
        shift-left: dbl[] [0.0, 0.0, 0.0, 1.0] -> [w356]
        tunnel: [w346] -> w29 mode=indexing
        shift-right: [w294] -> _
        shift-left: 0.0 -> [w301]
        shift-right: [w299] -> _
        shift-left: 0.0 -> [w302]
        shift-right: [w298] -> _
        shift-left: 0.0 -> [w303]
        shift-right: [w297] -> _
        shift-left: 0.0 -> [w304]
        shift-right: [w269] -> _
        shift-left: 0.0 -> [w273]
        shift-right: [w268] -> _
        shift-left: 0.0 -> [w272]
        shift-right: [w265] -> _
        shift-left: 0.0 -> [w271]
        shift-right: [w264] -> _
        shift-left: 0.0 -> [w270]
        i -> [w344]
        stop <- "STOP ALL" stop-if-true
        w363 = 0.01
        w314 = 30.7 ("input variable")
        w440 = 0.01
        # "Main Loop"
        n73 = case shown="True" "REINICIAR" {
          frame False {
          }
          frame True {
            (unwired) cluster{"e_th":dbl}[] [] ("History Data")
            (unwired) cluster{"e_d":dbl}[] [] ("History Data")
            n74 = property on="Lazo externo - Rumbo" class="WFChart (strict)"("History Data"=cluster{"x":dbl, "y":dbl}[] []) -> ()  [unwired: 2 in, 2 out]
            n75 = property on="Lazo externo - Posición" class="WFChart (strict)"("History Data"=cluster{"x":dbl, "y":dbl}[] []) -> ()  [unwired: 2 in, 2 out]
            n76 = property on="Señal de control de Velocidades" class="WFChart (strict)"("History Data"=cluster{"output":dbl, "output":dbl}[] []) -> ()  [unwired: 2 in, 2 out]
            n77 = property on="Desvio en Y (cm)" class="WFChart (strict)"("History Data"=cluster{"y":dbl}[] []) -> ()  [unwired: 2 in, 2 out]
            n78 = property on="Control Lazo Interno" class="WFChart (strict)"("History Data"=cluster{"f":dbl, dbl, "f":dbl, dbl}[] []) -> ()  [unwired: 2 in, 2 out]
          }
        }
        n79 = Or(x="REINICIAR", y=w277) -> (x .or. y?=w402:bool)
        n80 = Add(x="T pasa-bajos", y=w363) -> (x+y=w362:dbl)
        n81 = Divide(x=w363, y=w362) -> (x/y=w360:dbl)
        n82 = Add(x=w452, y=1.0) -> (x+y=w447:dbl)
        n83 = xnode ("Accelerometer")() -> ("X-Axis"=w368:dbl, "Y-Axis"=w366:dbl, "Z-Axis"=w365:dbl)  [unwired: 1 in, 1 out]
        n84 = xnode ("Encoder M1 Derecho")("Reset Counter"="REINICIAR") -> ("Counter Value"=w443:i32, "Counter Direction"=→"Dirección de Giro M1":T24)  [unwired: 1 in, 2 out]
        n85 = Wait Until Next ms Multiple(millisecond multiple=u32 10 ("milliseconds to wait")) -> ()  [unwired: 1 out]
        n86 = Negate(x=w443) -> (-x=w408:i32)
        "Cuentas M1 (Der)" <- w408
        n87 = Boolean To (0,1)(Boolean=w402) -> (0, 1=w394:i16)
        n88 = Multiply(x=3.141592653589793 ("Pi"), y=9.0) -> (x*y=w471:dbl)
        n89 = Divide(x=1440, y=w471) -> (x/y=w469:dbl)
        n90 = Divide(x=w408, y=w469) -> (x/y=w456:dbl)
        "Distancia  M1" <- w456
        n91 = Divide(x=w408, y=1440) -> (x/y=w464:dbl)
        "Vueltas Dadas M1" <- w464
        n92 = Multiply(x=w464, y=360.0) -> (x*y=→"Posición angular M1" →"Posición M1":dbl)
        n93 = call <vilib>:"Derivative x(t) PtByPt.vi"("initialize"=w402, "dt"=0.01, "initial condition"=0.0, "x"=w464) -> ("dx/dt"=w429:dbl)  [unwired: 1 out]
        n94 = Absolute Value(x=w429) -> (abs(x)=→"Frecuencia (rev/s)":dbl)
        n95 = Multiply(x=w429, y=60.0) -> (x*y=→"RPM M1" →"RPM GAUGE M1":dbl)
        n96 = Multiply(x=3.141592653589793 ("Pi"), y=9.0) -> (x*y=w465:dbl)
        n97 = Multiply(x=w465, y=w429) -> (x*y=w284:dbl)
        "Velocidad  M1" <- w284
        n98 = xnode ("Encoder M2 Izquierda")("Reset Counter"="REINICIAR") -> ("Counter Value"=w407:i32, "Counter Direction"=→"Dirección de Giro M2":T24)  [unwired: 1 in, 2 out]
        "Cuentas M2 (Izq)" <- w407
        n99 = Divide(x=w407, y=w469) -> (x/y=w454:dbl)
        "Distancia M2" <- w454
        n100 = Add(x=w456, y=w454) -> (x+y=w468:dbl)
        n101 = Divide(x=w468, y=2.0) -> (x/y=w379:dbl)
        "Recorrido Eje X (cm)" <- w379
        n102 = Equal?(x="MODO CONTROL", y=T13."Trayectoria" ("MODO CONTROL")) -> (x = y?=w382:bool)
        n103 = Not(x="REINICIAR") -> (.not. x?=w457:bool)
        n104 = Divide(x=w407, y=1440) -> (x/y=w463:dbl)
        "Vueltas Dadas M2" <- w463
        n105 = Select(t=w447, s="INICIAR MOTORES", f=0.0) -> (s? t:f=w446:dbl)
        n106 = Multiply(x=w463, y=360.0) -> (x*y=→"Posición angular M2" →"Posición M2":dbl)
        n107 = Not(x=w382) -> (.not. x?=w381:bool)
        n108 = call <vilib>:"Derivative x(t) PtByPt.vi"("initialize"=w402, "dt"=0.01, "initial condition"=0.0, "x"=w463) -> ("dx/dt"=w428:dbl)  [unwired: 1 out]
        n109 = Greater?(x=w379, y="Referencia M1 y M2") -> (0:w458:bool)
        n110 = To Double Precision Float(number="Movimiento") -> (double precision float=w292:dbl)
        n111 = Multiply(x=3.141592653589793 ("Pi"), y=9.0) -> (x*y=w460:dbl)
        n112 = Absolute Value(x=w428) -> (abs(x)=w475:dbl)
        n113 = Equal?(x="MODO CONTROL", y=T4."Lazo Interno" ("MODO CONTROL")) -> (x = y?=w413:bool)
        n114 = Multiply(x=w460, y=w428) -> (x*y=w283:dbl)
        "Velocidad M2" <- w283
        n115 = Add(x=w284, y=w283) -> (x+y=w375:dbl)
        n116 = Divide(x=w375, y=2.0) -> (x/y=w315:dbl)
        n117 = Subtract(x=w315, y=w373) -> (x-y=w370:dbl)
        n118 = Divide(x=w370, y=0.01) -> (x/y=w369:dbl)
        n119 = Divide(x=w369, y=981.0) -> (x/y=w367:dbl)
        "a_encoder" <- w367
        n120 = Build Array(w367, w368, w366, w365) -> (w361:dbl[])
        n121 = Subtract(x=w361, y=w356) -> (x-y=w345:dbl[])
        n122 = Multiply(x=w345, y=w360) -> (x*y=w359:dbl[])
        n123 = Add(x=w359, y=w356) -> (x+y=w357:dbl[])
        n124 = Index Array(array=w357) -> (element #1=w338:dbl, element #2=w354:dbl, element #3=w312:dbl, element #4=w353:dbl)  [unwired: 4 in]
        "a_enc_f" <- w338
        "aX_f" <- w354
        "aY_f" <- w312
        "aZ_f" <- w353
        n125 = formula code="float64 ah, ahr, z0, kspan, a, sg;\nfloat64 wz, z0r, kspan_r, ar, sr;\n\n// =====================================================================\n//  A) CORRECCIONES DINÁMICAS (aceleraciones del propio robot)\n// =====================================================================\n// Eje X: aceleración de avance (encoders) -> a_enc_f (ya filtrada)\n// Eje Y: aceleración centrípeta al girar avanzando\nwz    = (vR_med - vL_med)/L;                 // velocidad angular del robot (rad/s)\na_lat = V_med*wz/981;                        // centrípeta en Y (g)\n\naX_grav = aX_f - a_enc_f - Offset_acel;      // gravedad en X (sin aceleración ni offset)\naY_grav = aY_f - a_lat   - Offset_acelY;     // gravedad en Y (sin centrípeta ni offset)\n\n// =====================================================================\n//  B) PITCH (cabeceo: subir/bajar rampa, giro alrededor del eje Y)\n// =====================================================================\nah      = sqrt(aY_grav*aY_grav + aZ_f*aZ_f);\nphi     = atan2(aX_grav, ah);                // rad\nphi_deg = phi*180/3.14159265;                // grados\n\n// Calibración en dos puntos (de 8 ensayos: 2 en piso, 6 en rampa de 10°)\nz0    = 0.11;                                // cero: promedio de phi_deg en piso (°)\nkspan = 1.006;                               // span: 10° reales / 9.94° medidos\nphi_cal = kspan*(phi_deg - z0);\n\n// Zona muerta + saturación (grados)\na  = abs(phi_cal);\nsg = 1;\nif (phi_cal < 0) { sg = -1; }\nphi_lim = 0;\nphi_n   = 0;\nif (a > zm_deg) {\n    phi_lim = sg*min(a, ang_rampa);                                  // máx. ±ang_rampa\n    phi_n   = sg*min((a - zm_deg)/(ang_rampa - zm_deg), 1);          // -1 a 1\n}\n\n// =====================================================================\n//  C) ROLL (alabeo: ladeado a un costado, giro alrededor del eje X)\n// =====================================================================\nahr      = sqrt(aX_grav*aX_grav + aZ_f*aZ_f);\nroll     = atan2(aY_grav, ahr);              // rad\nroll_deg = roll*180/3.14159265;              // grados\n\n// Calibración en dos puntos  ->  VALORES PROVISIONALES (falta medirlos)\nz0r     = 0;                                 // cero del roll en piso (°)   -> de las pruebas A1/A2\nkspan_r = 1;                                 // span del roll               -> de las pruebas B1/B2\nroll_cal = kspan_r*(roll_deg - z0r);\n\n// Zona muerta + saturación (grados)\nar = abs(roll_cal);\nsr = 1;\nif (roll_cal < 0) { sr = -1; }\nroll_lim = 0;\nroll_n   = 0;\nif (ar > zm_deg) {\n    roll_lim = sr*min(ar, ang_rampa);\n    roll_n   = sr*min((ar - zm_deg)/(ang_rampa - zm_deg), 1);\n}" "Sintonización Acelerómetro"("aY_f"=w312, "a_enc_f"=w338, "aX_f"=w354, "aZ_f"=w353, "Offset_acel"="Offset acel_X", "zm_deg"="zona_muerta (°)", "ang_rampa"="ang_rampa", "Offset_acelY"="Offset_acel_Y", "vR_med"=w284, "vL_med"=w283, "V_med"=w315, "L"=w314) -> ("aX_grav"=w334:dbl, "phi"=w333:dbl, "phi_deg"=w321:dbl, "phi_cal"=w318:dbl, "phi_lim"=w305:dbl, "phi_n"=w317:dbl, "a_lat"=w311:dbl, "aY_grav"=w310:dbl, "roll_deg"=w309:dbl, "roll_cal"=w308:dbl, "roll_lim"=w307:dbl, "roll_n"=w306:dbl)  [unwired: 1 out]
        "aX_grav" <- w334
        "phi" <- w333
        "phi_deg" <- w321
        "Pitch - Eje Y" <- w318
        "Inclinación X" <- w305
        "pitch_n" <- w317
        "Inclinación Y" <- w307
        "roll_n" <- w306
        "Roll -  Eje X" <- w308
        n126 = formula code="float64 c = 0.019635;          // cm por cuenta = pi*9/1440\nfloat64 dsR, dsL, ds, dth;\n\nif (reset) {\n    x = 0;  y = 0;  th = 0;\n} else {\n    dsR = (cR - cR_ant)*c;     // avance de la rueda derecha [cm]\n    dsL = (cL - cL_ant)*c;     // avance de la rueda izquierda [cm]\n    ds  = (dsR + dsL)/2;       // avance del robot [cm]\n    dth = (dsR - dsL)/L;       // giro del robot [rad]\n    ds  = ds*cos(phi);         // proyección horizontal (rampa)\n    x  = x_ant + ds*cos(th_ant + dth/2);\n    y  = y_ant + ds*sin(th_ant + dth/2);\n    th = th_ant + dth;\n}\nth_deg = th*180/3.14159265;" "Cinemática Directa (Odometría)"("x_ant"=w427, "y_ant"=w358, "th_ant"=w426, "cR_ant"=w425, "cL_ant"=w424, "L"=w314, "phi"=w333, "reset"=w394, "cR"=w408, "cL"=w407) -> ("x"=w350:dbl, "y"=w340:dbl, "th"=w395:dbl, "th_deg"=w352:dbl)
        "X (cm)" <- w350
        "Y (cm)" <- w340
        "theta (deg)" <- w352
        n127 = formula code="float64 vc, wc, sg, eth, vR_raw, vL_raw, m, k;\nfloat64 tp, rf, dx, dy, dl, yl, listo, rut;\nfloat64 d1_p, giro_p, d2_p, d_iv, d1_r, giro_r, d2_r;\n\n// ===================== PARÁMETROS DE LAS RUTINAS =====================\n// Distancias en cm: POSITIVO = avanza, NEGATIVO = retrocede\n// Giros en grados:  POSITIVO = izquierda (antihorario), NEGATIVO = derecha\nd1_p = 100;   giro_p = 360;   d2_p = 100;      // tipo 4 RUTINA PISO : recta -> giro -> recta\nd_iv = 100;                                    // tipo 5 IDA Y VUELTA: avanza d_iv y retrocede d_iv\nd1_r = 230;   giro_r = 360;   d2_r = 230;      // tipo 6 RUTINA RAMPA: recta -> giro -> recta\n\n// ===================== ESTADO =====================\nvc = v;   wc = w;   sg = 1;   e_d = 0;   eth = 0;   listo = 0;\nfin  = fin_ant;   paso = paso_ant;\nx0 = x0_ant;   y0 = y0_ant;   th0 = th0_ant;\nif (reset != 0) { fin = 0; paso = 0; x0 = x; y0 = y; th0 = th; }\n\n// ===================== QUÉ TRAMO TOCA =====================\ntp = tipo;   rf = ref;   rut = 0;\nif (tipo == 4 || tipo == 5 || tipo == 6) {\n    rut = 1;\n    if (paso == 0) {                             // ---- TRAMO 1: recta ----\n        tp = 1;\n        rf = d1_p;\n        if (tipo == 5) { rf = d_iv; }\n        if (tipo == 6) { rf = d1_r; }\n    }\n    else if (paso == 1) {                        // ---- TRAMO 2: giro ----\n        tp = 2;\n        rf = giro_p;\n        if (tipo == 5) { rf = 0; }               // ida y vuelta: no gira (solo endereza el rumbo)\n        if (tipo == 6) { rf = giro_r; }\n    }\n    else if (paso == 2) {                        // ---- TRAMO 3: recta ----\n        tp = 1;\n        rf = d2_p;\n        if (tipo == 5) { rf = -d_iv; }           // ida y vuelta: retrocede lo mismo que avanzó\n        if (tipo == 6) { rf = d2_r; }\n    }\n    else { tp = 0; }                             // terminó\n}\n\n// posición medida desde el inicio del tramo\ndx = x - x0;   dy = y - y0;\ndl =  dx*cos(th0) + dy*sin(th0);                 // avance del tramo (+ adelante, - atrás)\nyl = -dx*sin(th0) + dy*cos(th0);                 // desvío lateral del tramo\n\nif (tp == 1) {                                   // ===== RECTA (avanza o retrocede) =====\n    e_d = rf - dl;\n    eth = th0 - th;\n    if (e_d < 0) { sg = -1; }                    // meta atrás -> retrocede\n    vc = Kd*e_d;\n    if (abs(vc) > vlim) { vc = sg*vlim; }\n    if (abs(vc) < vmin) { vc = sg*vmin; }\n    wc = Kth*eth - sg*Ky*yl;                     // en reversa la corrección lateral se invierte\n    wc = max(min(wc, 0.5), -0.5);\n    if (abs(e_d) < tol) { listo = 1; }\n}\nelse if (tp == 2 || tp == 3) {                   // ===== GIROS =====\n    eth = th0 + rf*3.14159265/180 - th;\n    if (eth < 0) { sg = -1; }\n    wc = Kth*eth;\n    if (abs(wc) > wlim) { wc = sg*wlim; }\n    if (abs(wc) < wmin) { wc = sg*wmin; }\n    vc = 0;\n    if (tp == 3) { vc = wc*L/2; }\n    if (abs(eth) < tol_th*3.14159265/180) { listo = 1; }\n}\n\n// ===================== AVANCE DEL GIRO =====================\n// se calcula ANTES de actualizar th0, para que el último valor sea el real\ngiro_deg = (th - th0)*180/3.14159265;            // cuánto ha girado en este tramo (°)\n\n// ===================== TRAMO TERMINADO =====================\nif (listo == 1) {\n    if (rut == 1) {                              // rutina: pasa al siguiente tramo\n        if (tp == 2 || tp == 3) { th0 = th0 + rf*3.14159265/180; }   // nuevo rumbo ideal\n        x0 = x;   y0 = y;\n        paso = paso + 1;\n    }\n    else { fin = 1; }                            // tipos 1-3: termina el ensayo\n}\nif (rut == 1 && paso >= 3) { fin = 1; }\nif (tipo > 0 && fin == 1) { vc = 0; wc = 0; }\ne_th = eth*180/3.14159265;\n\n// ===================== CINEMÁTICA INVERSA =====================\nvR_raw = vc + wc*L/2;\nvL_raw = vc - wc*L/2;\nm = max(abs(vR_raw), abs(vL_raw));\nk = 1;\nif (m > vmax) { k = vmax/m; }\nvR = k*vR_raw;\nvL = k*vL_raw;\n\n// ===================== SEÑALES PARA LAS GRÁFICAS =====================\nref_tramo = rf;                                  // referencia del tramo actual (cm o °)\navance    = dl;                                  // cuánto avanzó en este tramo (cm)\nrumbo_ref = th0*180/3.14159265;                  // rumbo deseado (°)\nif (tp == 2 || tp == 3) { rumbo_ref = (th0 + rf*3.14159265/180)*180/3.14159265; }\n\n// ===================== INDICADORES PARA EL PANEL =====================\nes_giro = 0;   es_recta = 0;\nif (tipo > 0 && fin == 0) {\n    if (tp == 2 || tp == 3) { es_giro = 1; }     // giro sobre centro o sobre rueda\n    if (tp == 1) { es_recta = 1; }               // recta (avanza o retrocede)\n}" "Cinemática Inversa"("v"="v(cm/s)", "w"="w (rad/s)", "L"=w314, "vmin"=3.0 ("input variable"), "tipo"="Movimiento", "ref"="Referencia", "x"=w350, "y"=w340, "th"=w395, "reset"=w394, "Kd"="Kd", "Kth"="Kth", "Ky"="Ky", "wmin"=0.3 ("input variable"), "tol"="Tolerancia (cm)", "tol_th"=1.0 ("input variable"), "vmax"=15.0 ("input variable"), "wlim"=0.4 ("input variable"), "vlim"=10.0 ("input variable"), "fin_ant"=w300, "paso_ant"=w301, "x0_ant"=w302, "y0_ant"=w303, "th0_ant"=w304) -> ("vR"=w355:dbl, "vL"=w376:dbl, "e_d"=w339:dbl, "e_th"=w291:dbl, "fin"=w388:dbl, "paso"=w294:dbl, "x0"=w299:dbl, "y0"=w298:dbl, "th0"=w297:dbl, "ref_tramo"=w260:dbl, "avance"=w296:dbl, "rumbo_ref"=w295:dbl, "giro_deg"=→"Giro Realizado (°)":dbl, "es_giro"=w259:dbl, "es_recta"=w258:dbl)
        "Error Distancia (cm)" <- w339
        "Error Ángulo (°)" <- w291
        n128 = Not Equal To 0?(x=w259) -> (x != 0?=→"Girando":bool)
        n129 = Not Equal To 0?(x=w258) -> (x != 0?=→"Avanzando":bool)
        n130 = Bundle("ref_tramo"=w260, "avance"=w296) -> (→"Lazo externo - Posición":cluster{"ref_tramo":dbl, "avance":dbl})  [unwired: 1 in]
        n131 = Select(t=w355, s=w382, f="Velocidad") -> (s? t:f=w418:dbl)
        n132 = Bundle("rumbo_ref"=w295, "th_deg"=w352) -> (→"Lazo externo - Rumbo":cluster{"rumbo_ref":dbl, "th_deg":dbl})  [unwired: 1 in]
        n133 = Select(t=w376, s=w382, f="Velocidad") -> (s? t:f=w416:dbl)
        n134 = Not Equal To 0?(x=w388) -> (x != 0?=w349:bool)
        "LLEGÓ" <- w349
        n135 = Boolean To (0,1)(Boolean=w349) -> (0, 1=w348:i16)
        n136 = Bundle("phi_lim"=w305, "roll_lim"=w307) -> (→"Comportamiento de ángulos (°)":cluster{"phi_lim":dbl, "roll_lim":dbl})  [unwired: 1 in]
        n137 = To Double Precision Float(number=w348) -> (double precision float=w347:dbl)
        n138 = Multiply(x=w475, y=60.0) -> (x*y=→"RPM GAUGE M2" →"RPM M2":dbl)
        n139 = To Double Precision Float(number=w344) -> (double precision float=w343:dbl)
        n140 = Or(x=w459, y=w458) -> (x .or. y?=w384:bool)
        n141 = Or(x=w413, y=w382) -> (x .or. y?=w287:bool)
        n142 = And(x=w384, y=w381) -> (x .and. y?=w383:bool)
        n143 = Multiply(x=w343, y=0.01) -> (x*y=w341:dbl)
        n144 = And(x=w383, y=w457) -> (x .and. y?=w449:bool)
        n145 = Boolean To (0,1)(Boolean="REINICIAR") -> (0, 1=w278:i16)
        n146 = Bundle("y"=w340) -> (→"Desvio en Y (cm)":cluster{"y":dbl})  [unwired: 1 in]
        n147 = Boolean To (0,1)(Boolean="INICIAR MOTORES") -> (0, 1=w323:i16)
        n148 = Greater Or Equal?(x=w446, y=50.0) -> (x >= y?=w444:bool)
        n149 = And(x=w444, y="INICIAR MOTORES") -> (x .and. y?=w445:bool)
        n150 = Not(x=w449) -> (.not. x?=w438:bool)
        n151 = And(x=w445, y=w438) -> (x .and. y?=w280:bool)
        n152 = Not(x=w280) -> (.not. x?=w404:bool)
        n153 = Or(x=w402, y=w404) -> (x .or. y?=w403:bool)
        n154 = Select(t="PWM Manual", s=w280, f=0.0) -> (s? t:f=w409:dbl)
        n155 = Select(t=w418, s=w280, f=0.0) -> (s? t:f=w285:dbl)
        n156 = call-poly <vilib>:"PID.vi"("reinitialize? (F)"=w403, "output range"=cluster{"output high":dbl, "output low":dbl} {"output high"=1.0, "output low"=-1.0}, "dt (s)"=0.01, "PID gains"="PI - M1", "process variable"=w284, "setpoint"=w285) -> ("output"=w336:dbl)  [unwired: 4 in, 1 out]
        n157 = Select(t=w416, s=w280, f=0.0) -> (s? t:f=w286:dbl)
        n158 = Bundle("f"=w285, w284, "f"=w286, w283) -> (→"Control Lazo Interno":cluster{"f":dbl, dbl, "f":dbl, dbl})  [unwired: 1 in]
        n159 = Boolean To (0,1)(Boolean=w280) -> (0, 1=w279:i16)
        n160 = call-poly <vilib>:"PID.vi"("reinitialize? (F)"=w403, "output range"="Rango Salida PWM", "dt (s)"=w440, "PID gains"="PI - M2", "process variable"=w283, "setpoint"=w286) -> ("output"=w335:dbl)  [unwired: 4 in, 1 out]
        n161 = formula code="float64 g_lim;\n\n// ===== FEEDFORWARD POR PENDIENTE (con ángulo limpio) =====\nff_R = 0;\nff_L = 0;\ng_lim = sin(phi_lim*3.14159265/180);      // pendiente limpia, en g (como aX_grav)\n\nif (run != 0 && abs(aX_grav) < 0.5 && phi_lim != 0) {\n    // motores ON + lectura razonable (< 30°) + fuera de la zona muerta (phi_lim ya trae 0 en piso)\n    if (g_lim > 0) {                       // SUBIENDO\n        ff_R = KgR_sub*g_lim;\n        ff_L = KgL_sub*g_lim;\n    } else {                               // BAJANDO\n        ff_R = KgR_baj*g_lim;\n        ff_L = KgL_baj*g_lim;\n    }\n}\n\nuR = max(min(uPI_R + ff_R, 1), -1);        // suma y satura entre -1 y 1\nuL = max(min(uPI_L + ff_L, 1), -1);" "FEED FORWARD - anticipar mov"("uPI_R"=w336, "uPI_L"=w335, "aX_grav"=w334, "KgR_sub"="KgR_sub", "KgL_sub"="KgL_sub", "KgR_baj"="KgR_baj", "KgL_baj"="KgL_baj", "run"=w323, "phi_lim"=w305) -> ("uR"=w326:dbl, "uL"=w325:dbl, "ff_R"=w328:dbl, "ff_L"=w327:dbl)
        "Aporte de FF-M1" <- w328
        "Aporte de FF-M2" <- w327
        n162 = Absolute Value(x=w326) -> (abs(x)=w288:dbl)
        n163 = Less Than 0?(x=w326) -> (x < 0?=w434:bool)
        n164 = Select(t=w288, s=w287, f=w409) -> (s? t:f=w401:dbl)
        n165 = Select(t=w434, s=w287, f=FALSE) -> (s? t:f=w290:bool)
        n166 = xnode ("DIO M1 Derecho")("DIR M1 (A/DIO0 (Pin 11))"=w290) -> ()  [unwired: 1 in, 1 out]
        n167 = Select(t=w401, s=w280, f=0.0) -> (s? t:f=w399:dbl)
        n168 = xnode ("PWM M1 Derecho")("Duty Cycle"=w399) -> ()  [unwired: 1 in, 1 out]
        n169 = formula code="float64 n_lim, v_ped, v_med;\nn_lim = 50;    // 50 vueltas x 10 ms = 0.5 s\nv_ped = 2.5;   // cm/s: se le pide moverse\nv_med = 0.5;   // cm/s: la rueda esta casi quieta\n\n// ===== AT SPEED (sigue la referencia) =====\natR = 0; atL = 0;\nif (arranque != 0 && abs(refR - velR) <= tol) { atR = 1; }\nif (arranque != 0 && abs(refL - velL) <= tol) { atL = 1; }\n\n// ===== FALLA (rueda trabada) =====\nnR = 0; nL = 0;\nif (arranque != 0 && abs(refR) >= v_ped && abs(velR) < v_med) { nR = nR_ant + 1; }\nif (arranque != 0 && abs(refL) >= v_ped && abs(velL) < v_med) { nL = nL_ant + 1; }\nif (nR > n_lim) { nR = n_lim; }\nif (nL > n_lim) { nL = n_lim; }\n\nfallaR = fR_ant; fallaL = fL_ant;\nif (nR >= n_lim) { fallaR = 1; }\nif (nL >= n_lim) { fallaL = 1; }\n\nif (reset != 0) { nR = 0; nL = 0; fallaR = 0; fallaL = 0; }"("refR"=w285, "velR"=w284, "refL"=w286, "velL"=w283, "tol"="Tol cm/s", "arranque"=w279, "reset"=w278, "nR_ant"=w273, "nL_ant"=w272, "fR_ant"=w271, "fL_ant"=w270) -> ("atR"=w275:dbl, "atL"=w274:dbl, "fallaR"=w265:dbl, "fallaL"=w264:dbl, "nR"=w269:dbl, "nL"=w268:dbl)
        n170 = Bundle("output"=w336, "output"=w335) -> (→"Señal de control de Velocidades":cluster{"output":dbl, "output":dbl})  [unwired: 1 in]
        n171 = Absolute Value(x=w325) -> (abs(x)=w412:dbl)
        n172 = Less Than 0?(x=w325) -> (x < 0?=w435:bool)
        n173 = Not(x=w435) -> (.not. x?=w432:bool)
        n174 = Build Array(w341, w347, "Referencia", w350, "Referencia", w352, w340, w285, w284, w336, w339, w286, w283, w335, w291, w338, w334, w321, w328, w327, w326, w325, w318, w305, w317, w312, w311, w310, w309, w308, w307, w306, w260, w296, w295, w294, w292) -> (w346:dbl[])
        n175 = Select(t=w412, s=w287, f=w409) -> (s? t:f=w397:dbl)
        n176 = Select(t=w397, s=w280, f=0.0) -> (s? t:f=w396:dbl)
        n177 = xnode ("PWM M2 Izquierda")("Duty Cycle"=w396) -> ()  [unwired: 1 in, 1 out]
        n178 = Not Equal To 0?(x=w275) -> (x != 0?=→"SIGUE Vel M1":bool)
        n179 = Not Equal To 0?(x=w274) -> (x != 0?=→"SIGUE Vel M2":bool)
        n180 = Not Equal To 0?(x=w264) -> (x != 0?=→"Falla M2":bool)
        n181 = Select(t=w432, s=w287, f=TRUE) -> (s? t:f=w430:bool)
        n182 = Not Equal To 0?(x=w265) -> (x != 0?=→"Falla M1":bool)
        n183 = xnode ("DIO M2 Izquierda")("DIR M2 (B/DIO0 (Pin 11))"=w430) -> ()  [unwired: 1 in, 1 out]
        "Móvil dt" <- w440
      }
    }
    frame #2 {
      w780 = path "/home/lvuser/control_balanceo_13_11" ("file path (dialog if empty)")
      w792 = path "/home/lvuser/control_movil_13_girocorregido" ("file path (dialog if empty)")
      # "Close"
      n184 = xnode ("PWM M2 Izquierda")("Duty Cycle"=0.0) -> ()  [unwired: 1 in, 1 out]
      n185 = xnode ("PWM M1 Derecha")("Duty Cycle"=0.0) -> ()  [unwired: 1 in, 1 out]
      n186 = call <vilib>:"Reset myRIO.vi"("error in (no error)"=w802) -> ()  [unwired: 10 in, 1 out]
      n187 = VISA Close(VISA resource name=w770, error in (no error)=w771) -> (error out=w772:errorcluster)
      n188 = xnode ("PWM Servo EjeY")("Duty Cycle"=0.0) -> ()  [unwired: 1 in, 1 out]
      n189 = Open/Create/Replace File(file path (use dialog)=w780, operation (0:open)=T23."replace or create") -> (refnum out=w776:refnum<file>, error out=w778:errorcluster)  [unwired: 4 in, 1 out]
      n190 = xnode ("PWM Servo EjeX")("Duty Cycle"=0.0) -> ()  [unwired: 1 in, 1 out]
      n191 = Open/Create/Replace File(file path (use dialog)=w792, operation (0:open)=T23."replace or create") -> (refnum out=w788:refnum<file>, error out=w790:errorcluster)  [unwired: 4 in, 1 out]
      n192 = call <vilib>:"Reset myRIO.vi"("error in (no error)"=w772) -> ("error out"=→"error out 2":errorcluster)  [unwired: 10 in]
      n193 = local write "STOP ALL"(FALSE ("STOP ALL")) -> ()
      n194 = Write to Text File(file (use dialog)=w776, text="inclinacion_x,x,erro_x,inclinacion_y,y,error_y\n", error in=w778) -> (error out=w777:errorcluster)  [unwired: 1 in, 2 out]
      n195 = Close File(refnum=w776, error in=w777) -> (error out=w775:errorcluster)  [unwired: 1 out]
      n196 = call-poly <vilib>:"Write Delimited Spreadsheet.vi"("file path (dialog if empty)"=w780, "format (%.3f)"="%.6f", "2D data"=w774, "append to file? (new file:F)"=TRUE, "error in (no error)"=w775, "delimiter (\\t)"="," ("delimiter (\\t)")) -> ("error out"=→"Verifica si se guardo csv 2":errorcluster)  [unwired: 8 in, 1 out]
      n197 = Write to Text File(file (use dialog)=w788, text="t,llego,ref_recta,x_odo,ref,th_deg_odo,y_odo,SpVel_M1,Vel_M1,u_M1,error_distancia,SpVel_M2,Vel_M2,u_M2,error_angular,a_enc_f,aX_grav,phi_deg,ff_R,ff_L,uR,uL,phi_cal,phi_lim,phi_n,aY_f,a_lat,aY_grav,roll_deg,roll_cal,roll_lim,roll_n,ref_tramo,avance,rumbo_ref,paso,tipo\n", error in=w790) -> (error out=w789:errorcluster)  [unwired: 1 in, 2 out]
      n198 = Close File(refnum=w788, error in=w789) -> (error out=w787:errorcluster)  [unwired: 1 out]
      n199 = call-poly <vilib>:"Write Delimited Spreadsheet.vi"("file path (dialog if empty)"=w792, "format (%.3f)"="%.6f", "2D data"=w786, "append to file? (new file:F)"=TRUE, "error in (no error)"=w787, "delimiter (\\t)"="," ("delimiter (\\t)")) -> ("error out"=→"Verifica si se guardo csv":errorcluster)  [unwired: 8 in, 1 out]
    }
  }
